vi "Q17_Two_Plots.vi"() -> ()   [LabVIEW 2018]
doc: "Use this template to build a VI to use as a subVI."
panel:
  out "D":dbl[][](array[numeric])
  out "C (insert sine 5 at row 0)":dbl[][](array[numeric])
  out "B":dbl[][](array[numeric])
  out "A":dbl[](array[numeric])
  in  "Sine 1":dbl[](array[numeric])
  in  "Sine 5":dbl[](array[numeric])
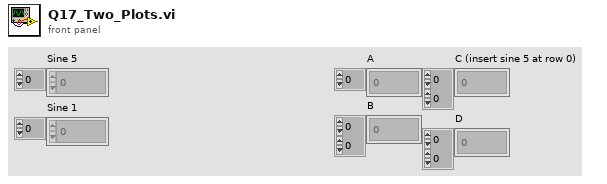
[diagram p1: front panel]
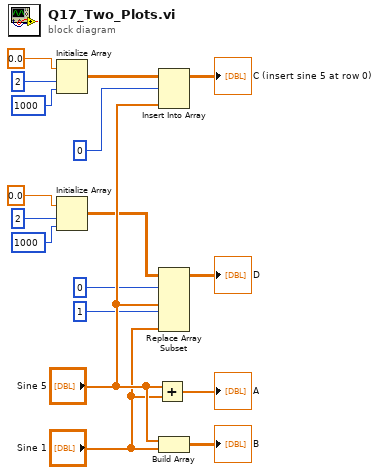
[diagram p0: block diagram]
diagram:
  n1 = Initialize Array(0.0 ("element"), 2 ("dimension size"), 1000 ("dimension size")) -> (w10:dbl[][])
  n2 = Initialize Array(0.0 ("element"), 2 ("dimension size"), 1000 ("dimension size")) -> (w4:dbl[][])
  n3 = Add(x="Sine 5", y="Sine 1") -> (x+y=→"A":dbl[])
  n4 = Insert Into Array(array=w10, index (row)=0, new element="Sine 5") -> (→"C (insert sine 5 at row 0)":dbl[][])  [unwired: 1 in]
  n5 = Replace Array Subset(array=w4, new element #1="Sine 5", index (row) #1=0 ("index (row)"), new element #2="Sine 1", index (row) #2=1 ("index (row)")) -> (→"D":dbl[][])  [unwired: 2 in]
  n6 = Build Array("Sine 5", "Sine 1") -> (→"B":dbl[][])
